vi "Get State String Info.vi"(8 "error in (no error)":errorcluster, 10 "GObj Refnum in":refnum<vi>, 11 "JKI SM in":refnum<class "JKI SM.lvclass">) -> (0 "error out":errorcluster, 1 "Frame Name":string, 2 "Structure":string, 3 "JKI SM out":refnum<class "JKI SM.lvclass">)   [LabVIEW 2020, in "JKI State Machine API.lvlib" / "JKI SM.lvclass"]
uses:
  JKI SM.lvclass
  JKI SM.lvclass/JKI SM.ctl
panel:
  out "Class Name":string
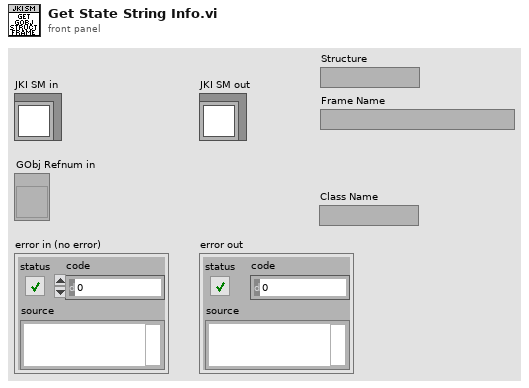
[diagram p1: front panel]
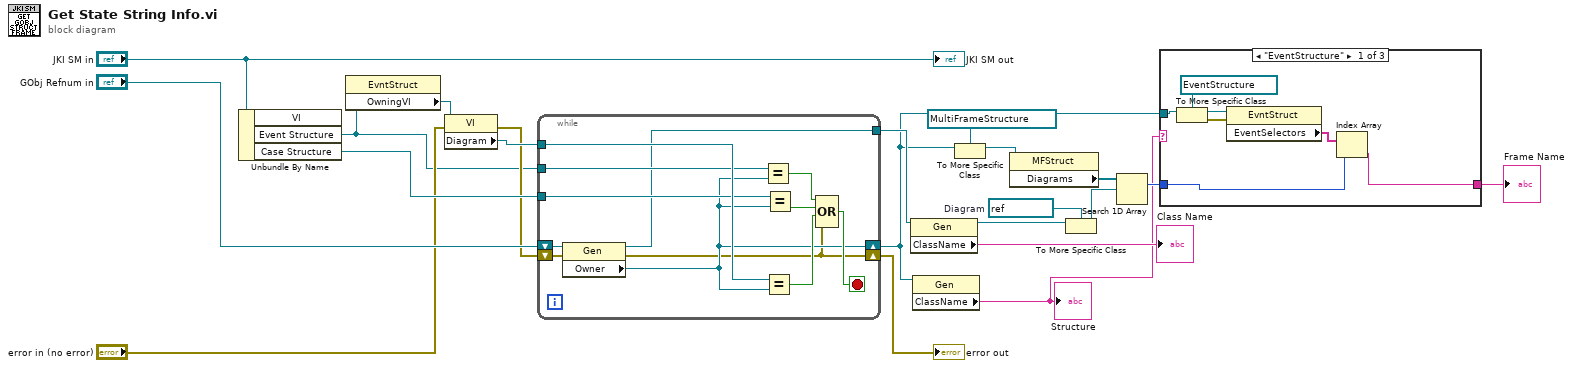
[diagram p0: block diagram]
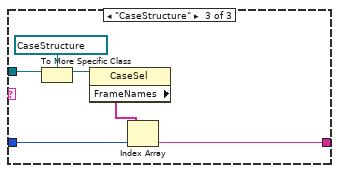
[diagram p3: hidden frame]
diagram:
  w11 = refnum<vi> refnum  # Diagram
  n1 = Unbundle By Name("JKI SM in") -> ("Event Structure"=w6:refnum<vi>, "Case Structure"=w18:refnum<vi>)  [unwired: 1 out]
  n2 = property class="EvntStruct"(reference=w6) -> ("OwningVI"=w5:refnum<vi>)  [unwired: 1 in, 2 out]
  n3 = property class="VI"(reference=w5, error in="error in (no error)") -> (error out=w15:errorcluster, "Diagram"=w19:refnum<vi>)  [unwired: 1 out]
  n4 = while {
    shift-right: [w25] -> w3
    shift-left: "GObj Refnum in" -> [w33]
    tunnel: w19 -> [w32]
    tunnel: w6 -> [w31]
    tunnel: w18 -> [w27]
    tunnel: [w24] -> w16
    shift-right: [w22] -> w13
    shift-left: w15 -> [w23]
    stop <- w28 stop-if-true
    n5 = property class="Gen"(reference=w33, error in=w23) -> (reference out=w24:refnum<vi>, error out=w22:errorcluster, "Owner"=w25:refnum<vi>)
    n6 = Equal?(x=w31, y=w25) -> (x = y?=w30:bool)
    n7 = Equal?(x=w32, y=w25) -> (x = y?=w29:bool)
    n8 = Equal?(x=w27, y=w25) -> (x = y?=w26:bool)
    n9 = Compound Arithmetic op=OR(w30, w26, w29, w22) -> (w28:bool)
  }
  "error out" <- w13
  n10 = property class="Gen"(reference=w16) -> (reference out=w10:refnum<vi>, "ClassName"=→"Class Name":string)  [unwired: 1 in, 1 out]
  n11 = property class="Gen"(reference=w3) -> ("ClassName"=w1:string)  [unwired: 1 in, 2 out]
  "Structure" <- w1
  n12 = To More Specific Class(target class=refnum<vi> refnum ("Part References.Case Structure"), reference=w3) -> (specific class reference=w2:refnum<vi>)  [unwired: 1 in, 1 out]
  n13 = property class="MFStruct"(reference=w2) -> ("Diagrams"=w12:refnum<vi>[])  [unwired: 1 in, 2 out]
  n14 = To More Specific Class(target class=w11, reference=w10) -> (specific class reference=w9:refnum<vi>)  [unwired: 1 in, 1 out]
  n15 = Search 1D Array(1D array=w12, element=w9) -> (index of element=w8:i32)  [unwired: 1 in]
  n16 = case shown="\"EventStructure\"" w1 {
    tunnel: w8 -> [w35 _ w45]
    tunnel: [w34 _ w44] -> w7
    tunnel: w3 -> [w40 _ w41]
    frame "EventStructure" {
      n17 = To More Specific Class(target class=refnum<vi> refnum ("Part References.Case Structure"), reference=w40) -> (specific class reference=w38:refnum<vi>, error out=w37:errorcluster)  [unwired: 1 in]
      n18 = property class="EvntStruct"(reference=w38, error in=w37) -> ("EventSelectors"=w36:string[])  [unwired: 2 out]
      n19 = Index Array(array=w36, index=w35) -> (element=w34:string)
    }
    frame Default {
    }
    frame "CaseStructure" {
      n20 = To More Specific Class(target class=refnum<vi> refnum ("Part References.Case Structure"), reference=w41) -> (specific class reference=w43:refnum<vi>)  [unwired: 1 in, 1 out]
      n21 = property class="CaseSel"(reference=w43) -> ("FrameNames"=w42:string[])  [unwired: 1 in, 2 out]
      n22 = Index Array(array=w42, index=w45) -> (element=w44:string)
    }
  }
  "Frame Name" <- w7
  "JKI SM out" <- "JKI SM in"
